vi "Test_API_Receive.vi"() -> ()   [LabVIEW 2021]
doc: "A4 test: S4 through the API (Init, Frames_Create, Open, loop {Read ? Frame_Get}, Status, Close). Also tests the Lost path when the WebSocket is closed from outside."
uses:
  api/CANsub_Channel/CANsub_Channel.lvclass
  typedefs/Test_RX_Stats.ctl
  common/Typedefs/CANsub_connection.ctl
  common/CANsub_Common.lvlib
  common/Typedefs/CANsub_Bit_Rates.ctl
  api/Typedefs/CANsub_Filter.ctl
  api/CANsub_API.lvlib
  api/Typedefs/CANsub_Read_Mode.ctl
  api/Typedefs/CANsub_Ownership.ctl
  api/Typedefs/CANsub_Config.ctl
  api/Typedefs/CANsub_State.ctl
  common/Typedefs/Bit_Timing.ctl
  api/Typedefs/CANsub_Status.ctl
panel:
  in  "read timeout ms":i32=100
  in  "run time (sec)":u32=30
  out "error out":errorcluster
  out "status":T1
  out "stats":T4 {"last data" format="%.0x"; "ids" format="%.0x"}
  in  "config":T5={"connection"={"host"="192.168.0.49", "channel"=2, "cert path"=path "/home/lvuser/cansub_root_cert.crt"}, "bit rates"={"nominal bit rate"=500000, "nominal sample point"=80.0, "data bit rate"=2000000, "data sample point"=80.0}, "listen only"=FALSE, "filters"=[], "read mode"=enum."Poll", "max bytes per read"=4096, "reader FIFO depth"=0, "reader priority"=0, "ownership"=enum."Direct"} {"filters"."f2" format="%.0x"; "filters"."f1" format="%.0x"}
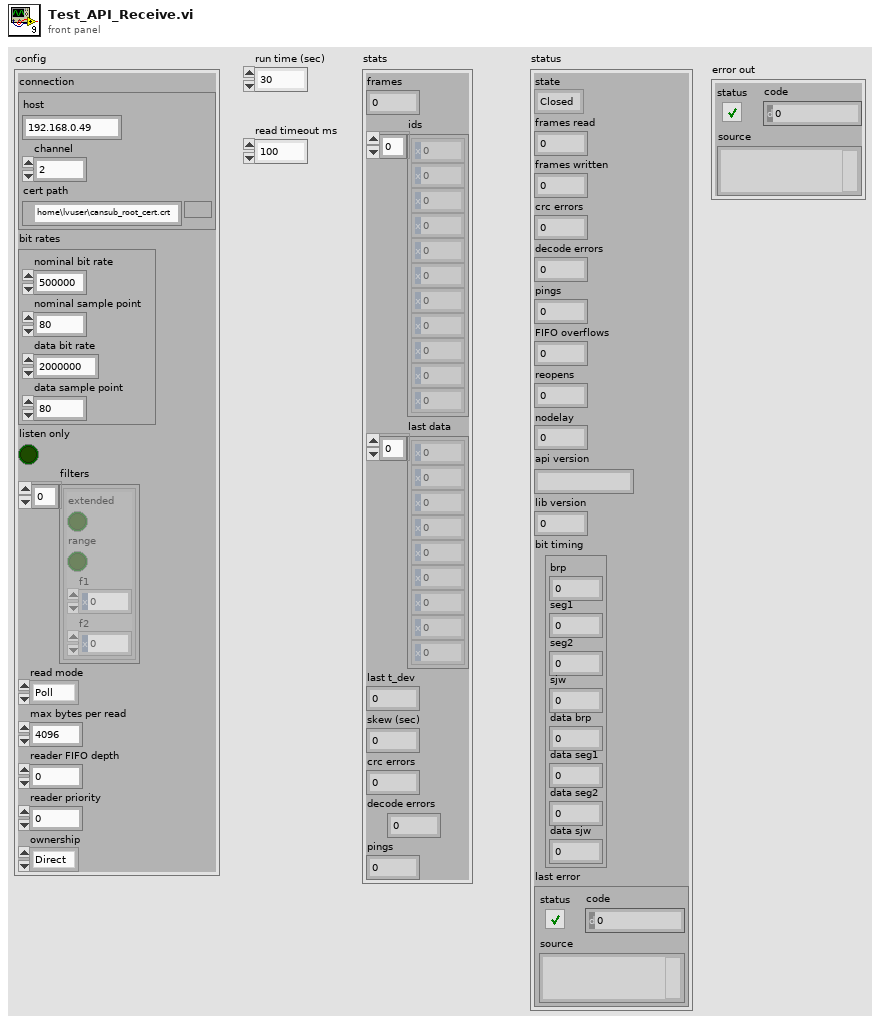
[diagram p1: front panel]
types:
  T1 = typedef "CANsub_API.lvlib/CANsub_Status.ctl" = cluster{"state":T2, "frames read":u32, "frames written":u32, "crc errors":u32, "decode errors":i32, "pings":u32, "FIFO overflows":u32, "reopens":u32, "nodelay":i32, "api version":string, "lib version":u32, "bit timing":T3, "last error":errorcluster}
  T2 = typedef "CANsub_API.lvlib/CANsub_State.ctl" = enum16{"Closed", "Open", "Lost"}
  T3 = typedef "CANsub_Common.lvlib/Bit_Timing.ctl" = cluster{"brp":u16, "seg1":u16, "seg2":u16, "sjw":u16, "data brp":u16, "data seg1":u16, "data seg2":u16, "data sjw":u16}
  T4 = typedef "Test_RX_Stats.ctl" = cluster{"frames":i32, "ids":u32[], "last data":u8[], "last t_dev":dbl, "skew (sec)":dbl, "crc errors":u32, "decode errors":i32, "pings":i32}
  T5 = typedef "CANsub_API.lvlib/CANsub_Config.ctl" = cluster{"connection":T6, "bit rates":T7, "listen only":bool, "filters":T8[], "read mode":T9, "max bytes per read":i32, "reader FIFO depth":i32, "reader priority":i32, "ownership":T10}
  T6 = typedef "CANsub_Common.lvlib/CANsub_connection.ctl" = cluster{"host":string, "channel":u8, "cert path":path}
  T7 = typedef "CANsub_Common.lvlib/CANsub_Bit_Rates.ctl" = cluster{"nominal bit rate":u32, "nominal sample point":dbl, "data bit rate":u32, "data sample point":dbl}
  T8 = typedef "CANsub_API.lvlib/CANsub_Filter.ctl" = cluster{"extended":bool, "range":bool, "f1":u32, "f2":u32}
  T9 = typedef "CANsub_API.lvlib/CANsub_Read_Mode.ctl" = enum16{"Poll", "Reader"}
  T10 = typedef "CANsub_API.lvlib/CANsub_Ownership.ctl" = enum16{"Direct", "Shared"}
  T11 = typedef "CANsub_API.lvlib/CANsub_Frames.ctl" = cluster{"count":i32, "t_dev":dbl[], "id":u32[], "flags":u16[], "dlc":u8[], "data len":u8[], "data":u8[]}
  T12 = typedef "CANsub_API.lvlib/CANsub_Frame.ctl" = cluster{"id":u32, "t_dev":dbl, "dlc":u8, "data len":u8, "ide":bool, "fdf":bool, "rtr":bool, "brs":bool, "esi":bool, "tx ack":bool, "error frame":bool}
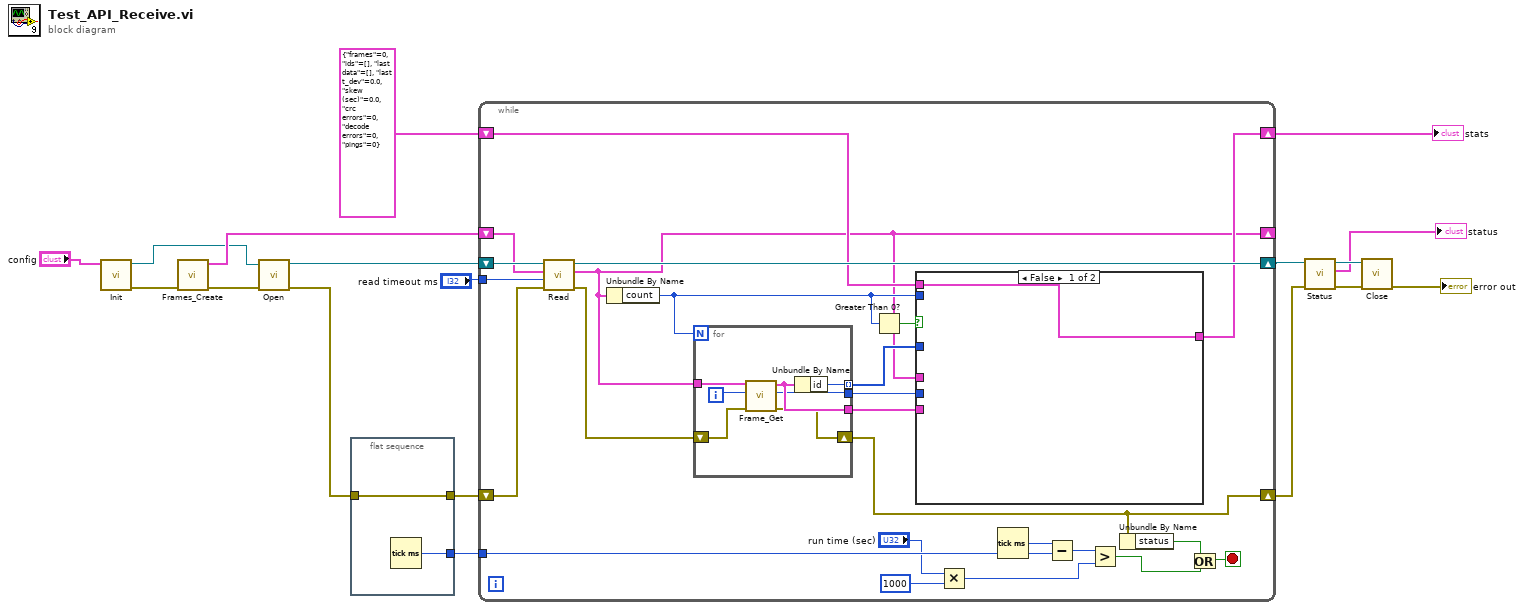
[diagram p0: block diagram]
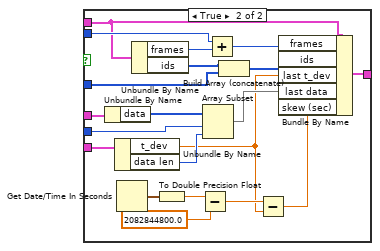
[diagram p2: hidden frame]
diagram:
  n1 = call "Init.vi"("config"="config") -> ("error out"=w17:errorcluster, "channel out"=w6:refnum<class "CANsub_Channel.lvclass">)  [unwired: 8 in, 1 out]
  n2 = call "Frames_Create.vi"("error in (no error)"=w17) -> ("error out"=w16:errorcluster, "frames"=w12:T11)  [unwired: 9 in]
  n3 = call-dynamic "Open.vi"("error in (no error)"=w16, "channel in"=w6) -> ("error out"=w15:errorcluster, "channel out"=w13:refnum<class "CANsub_Channel.lvclass">)  [unwired: 8 in]
  n4 = flat-sequence {
    tunnel: w15 -> [w19]
    tunnel: [w20] -> w7
    tunnel: [w19] -> w14
    frame #0 {
      n5 = Tick Count (ms)() -> (millisecond timer value=w20:u32)
    }
  }
  n6 = while {
    shift-right: [w22] -> w5
    shift-left: w14 -> [w40]
    shift-right: [w36] -> w8
    shift-left: T4 {"frames"=0, "ids"=[], "last data"=[], "last t_dev"=0.0, "skew (sec)"=0.0, "crc errors"=0, "decode errors"=0, "pings"=0} ("stats") -> [w37]
    shift-right: [w32] -> _
    shift-left: w12 -> [w43]
    shift-right: [w41] -> w3
    shift-left: w13 -> [w44]
    tunnel: "read timeout ms" -> [w42]
    tunnel: w7 -> [w29]
    stop <- w21 stop-if-true
    n7 = call-dynamic "Read.vi"("error in (no error)"=w40, "timeout ms"=w42, "frames in"=w43, "channel in"=w44) -> ("error out"=w39:errorcluster, "frames out"=w32:T11, "channel out"=w41:refnum<class "CANsub_Channel.lvclass">)  [unwired: 5 in]
    n8 = Unbundle By Name(w32) -> ("count"=w34:i32)
    n9 = for {
      N: w34 -> [_]
      tunnel: w32 -> [w72]
      tunnel: [w70] -> w35 mode=indexing
      tunnel: [w69] -> w33
      tunnel: [w68] -> w31
      shift-right: [w66] -> w22
      shift-left: w39 -> [w67]
      i -> [w71]
      n10 = call "Frame_Get.vi"("error in (no error)"=w67, "i"=w71, "frames"=w72) -> ("error out"=w66:errorcluster, "data offset"=w68:i32, "frame"=w69:T12)  [unwired: 6 in]
      n11 = Unbundle By Name(w69) -> ("id"=w70:u32)
    }
    n12 = Greater Than 0?(x=w34) -> (x > 0?=w38:bool)
    n13 = case shown="False" w38 {
      tunnel: w37 -> [w45 w57]
      tunnel: [w45 w58] -> w36
      tunnel: w35 -> [_ w64]
      tunnel: w34 -> [_ w62]
      tunnel: w33 -> [_ w61]
      tunnel: w32 -> [_ w56]
      tunnel: w31 -> [_ w54]
      frame False {
      }
      frame True {
        n14 = Unbundle By Name(w56) -> ("data"=w55:u8[])
        n15 = Unbundle By Name(w61) -> ("t_dev"=w47:dbl, "data len"=w53:u8)
        n16 = Get Date/Time In Seconds() -> (seconds since 1Jan1904=w51:timestamp)
        n17 = Unbundle By Name(w57) -> ("frames"=w63:i32, "ids"=w65:u32[])
        n18 = To Double Precision Float(number=w51) -> (double precision float=w50:dbl)
        n19 = Subtract(x=w50, y=2082844800.0) -> (x-y=w48:dbl)
        n20 = Array Subset(array=w55, index=w54, length=w53) -> (w52:u8[])
        n21 = Add(x=w62, y=w63) -> (x+y=w60:i32)
        n22 = Build Array (concatenate)(w65, w64) -> (w59:u32[])
        n23 = Subtract(x=w48, y=w47) -> (x-y=w46:dbl)
        n24 = Bundle By Name(cluster=w57, "frames"=w60, "ids"=w59, "last t_dev"=w47, "last data"=w52, "skew (sec)"=w46) -> (w58:T4)
      }
    }
    n25 = Multiply(x="run time (sec)", y=u32 1000) -> (x*y=w25:u32)
    n26 = Tick Count (ms)() -> (millisecond timer value=w30:u32)
    n27 = Subtract(x=w30, y=w29) -> (x-y=w28:u32)
    n28 = Greater?(x=w28, y=w25) -> (0:w23:bool)
    n29 = Unbundle By Name(w22) -> ("status"=w24:bool)
    n30 = Or(x=w24, y=w23) -> (x .or. y?=w21:bool)
  }
  "stats" <- w8
  n31 = call-dynamic "Status.vi"("error in (no error)"=w5, "channel in"=w3) -> ("error out"=w4:errorcluster, "status"=→"status":T1, "channel out"=w2:refnum<class "CANsub_Channel.lvclass">)  [unwired: 7 in]
  n32 = call-dynamic "Close.vi"("error in (no error)"=w4, "channel in"=w2) -> ("error out"=→"error out":errorcluster)  [unwired: 8 in, 1 out]
